vi "locate engine.vi"(8 "error in":errorcluster, 11 "component":T1) -> (0 "error out":errorcluster, 3 "engine":refnum<data-value>)   [LabVIEW 2013, in "PL Framework Configuration Tool.lvlib" / "module editor node.lvclass"]
uses:
  module editor node.lvclass
  Engine Parent/Engine Parent Editor Node.lvclass
  <vilib>/NI/Configuration Framework/Node/NodeRef.ctl
  <vilib>/NI/Configuration Framework/Node/NISE_CEF_Node.lvclass
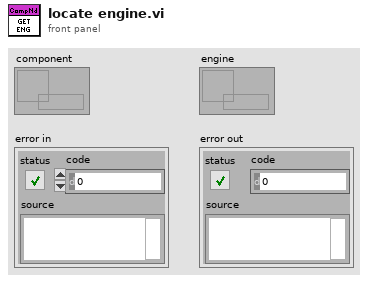
[diagram p1: front panel]
types:
  T1 = typedef "NISE_CEF_Node.lvclass/NodeRef.ctl" = refnum<data-value>
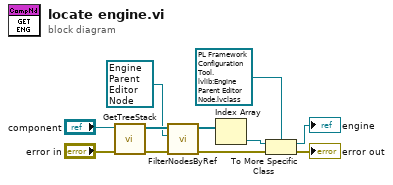
[diagram p0: block diagram]
diagram:
  n1 = call <vilib>:"GetTreeStack.vi"("error in"="error in", "node in"="component") -> ("error out"=w8:errorcluster, "parents"=w9:refnum<data-value>[])  [unwired: 8 in]
  n2 = call <vilib>:"FilterNodesByRef.vi"("error in"=w8, "NISE_CEF_Node"=refnum<class "Engine Parent Editor Node.lvclass"> refnum ("PL Framework Configuration Tool.lvlib:Engine Parent Editor Node.lvclass"), "nodes"=w9) -> ("error out"=w5:errorcluster, "filtered nodes"=w6:refnum<data-value>[])  [unwired: 7 in]
  n3 = Index Array(array=w6) -> (element=w3:refnum<data-value>)  [unwired: 1 in]
  n4 = To More Specific Class(target class=refnum<data-value> refnum, reference=w3, error in=w5) -> (specific class reference=→"engine":refnum<data-value>, error out=→"error out":errorcluster)
